vi "bats.parser.generated.vi"(9 "time":u64, 10 "data.stream":T1={"data"=[0, 0, 0, 0, 0, 0, 0, 0], "data valid"=FALSE, "byte enables"=[FALSE, FALSE, FALSE, FALSE, FALSE, FALSE, FALSE, FALSE], "eof.good"=FALSE, "eof.bad"=FALSE, "recv.time"=0}, 11 "reset":bool) -> (2 "Ready.for.Udp.Input":bool)   [LabVIEW 2020]
doc: "REFERENCE COPY of bats.parser.vi, built 2026-10-14 from its AIXML export. The two FPGA FIFO Write nodes (handshake interface), which AIXML cannot carry, are replaced by calls to FIFO.WRITE.vi with the FIFO's configuration wired as constants: FIFO Name and Data Type, Element through To Variant. Everything else is the exported diagram; typedefs come back as bare clusters (rebind if this is ever used for real). To put the real FIFO nodes back: replace each FIFO.WRITE.vi call with the FPGA FIFO Method Node (Write) for the named FIFO, wire Element and Input Valid, read Ready for Input, delete the constants and To Variant."
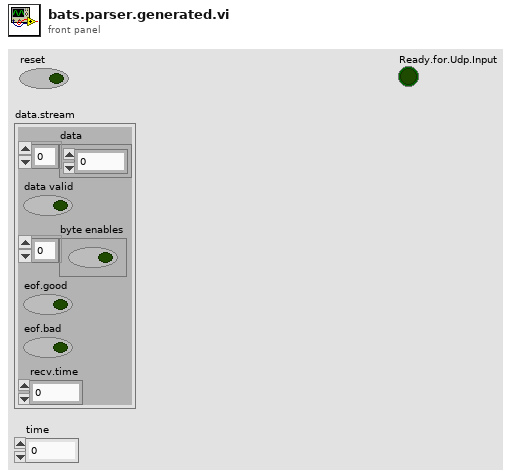
[diagram p1: front panel]
types:
  T1 = cluster{"data":u8[], "data valid":bool, "byte enables":bool[], "eof.good":bool, "eof.bad":bool, "recv.time":u64}
  T2 = cluster{"reset":bool, "data.stream":cluster{"data":u8[], "data valid":bool, "byte enables":bool[], "eof.good":bool, "eof.bad":bool, "recv.time":u64}}
  T3 = enum16{"Reset", "Noop", "Read.Sequenced.Unit.Header", "Read.Msg"}
  T4 = cluster{"BATS.Parser.States":enum16{"Reset", "Noop", "Read.Sequenced.Unit.Header", "Read.Msg"}, "Saved.BATS.Parser.State":enum16{"Reset", "Noop", "Read.Sequenced.Unit.Header", "Read.Msg"}, "Hdr Length (U16)":u16, "MessageLength (U8)":u8, "MessageType (U8)":u8, "Time (U32)":u32, "Total Counter (U16)":u16, "Message Counter (U8)":u8, "i":u16, "Number.of.Tickers":u16, "n":u16, "msg.counter":u8, "msg.length":u8, "buffer.start":u8, "buffer.length":u8, "buffer":u64[], "Next.Seq.No":u32, "debug":cluster{"write":bool, "data":u64[]}}
  T5 = enum8{"Time", "AddOrder", "OrderExecuted", "OrderExecutedAtPrice", "ReduceSize", "ModifyOrder", "DeleteOrder", "Get.Everything", "Get.All.Orders", "Get.Top", "Trade", "Unsupported"}
  T6 = cluster{"type":enum8{"Time", "AddOrder", "OrderExecuted", "OrderExecutedAtPrice", "ReduceSize", "ModifyOrder", "DeleteOrder", "Get.Everything", "Get.All.Orders", "Get.Top", "Trade", "Unsupported"}, "side":u8, "orderId ":u64, "quantity":u32, "symbol":u64, "price":u64, "executed.qty":u32, "canceled.qty":u32, "remaining.qty":u32, "seconds":u64, "nanoseconds":u64, "Add":bool, "Edit":bool, "Remove":bool, "seq no":u32, "recv.time":u64, "parse.time":u64}
  T7 = typedef "fpganow.common.fpga.lvlib/orderbook.command.ctl" = cluster{"type":T8, "side":u8, "orderId ":u64, "quantity":u32, "symbol":u64, "price":u64, "executed.qty":u32, "canceled.qty":u32, "remaining.qty":u32, "seconds":u64, "nanoseconds":u64, "Add":bool, "Edit":bool, "Remove":bool, "seq no":u32, "recv.time":u64, "parse.time":u64}
  T8 = typedef "fpganow.common.fpga.lvlib/orderbook.command.type.ctl" = enum8{"Time", "AddOrder", "OrderExecuted", "OrderExecutedAtPrice", "ReduceSize", "ModifyOrder", "DeleteOrder", "Get.Everything", "Get.All.Orders", "Get.Top", "Trade", "Unsupported"}
  T9 = cluster{"type":enum8{"Time", "AddOrder", "OrderExecuted", "OrderExecutedAtPrice", "ReduceSize", "ModifyOrder", "DeleteOrder", "Get.Everything", "Get.All.Orders", "Get.Top"}, "side":u8, "orderId ":u64, "quantity":u32, "symbol":u64, "price":u64, "executed.qty":u32, "canceled.qty":u32, "remaining.qty":u32, "seconds":u64, "nanoseconds":u64, "Add":bool, "Edit":bool, "Remove":bool, "seq no":u32, "recv.time":u64, "parse.time":u64}
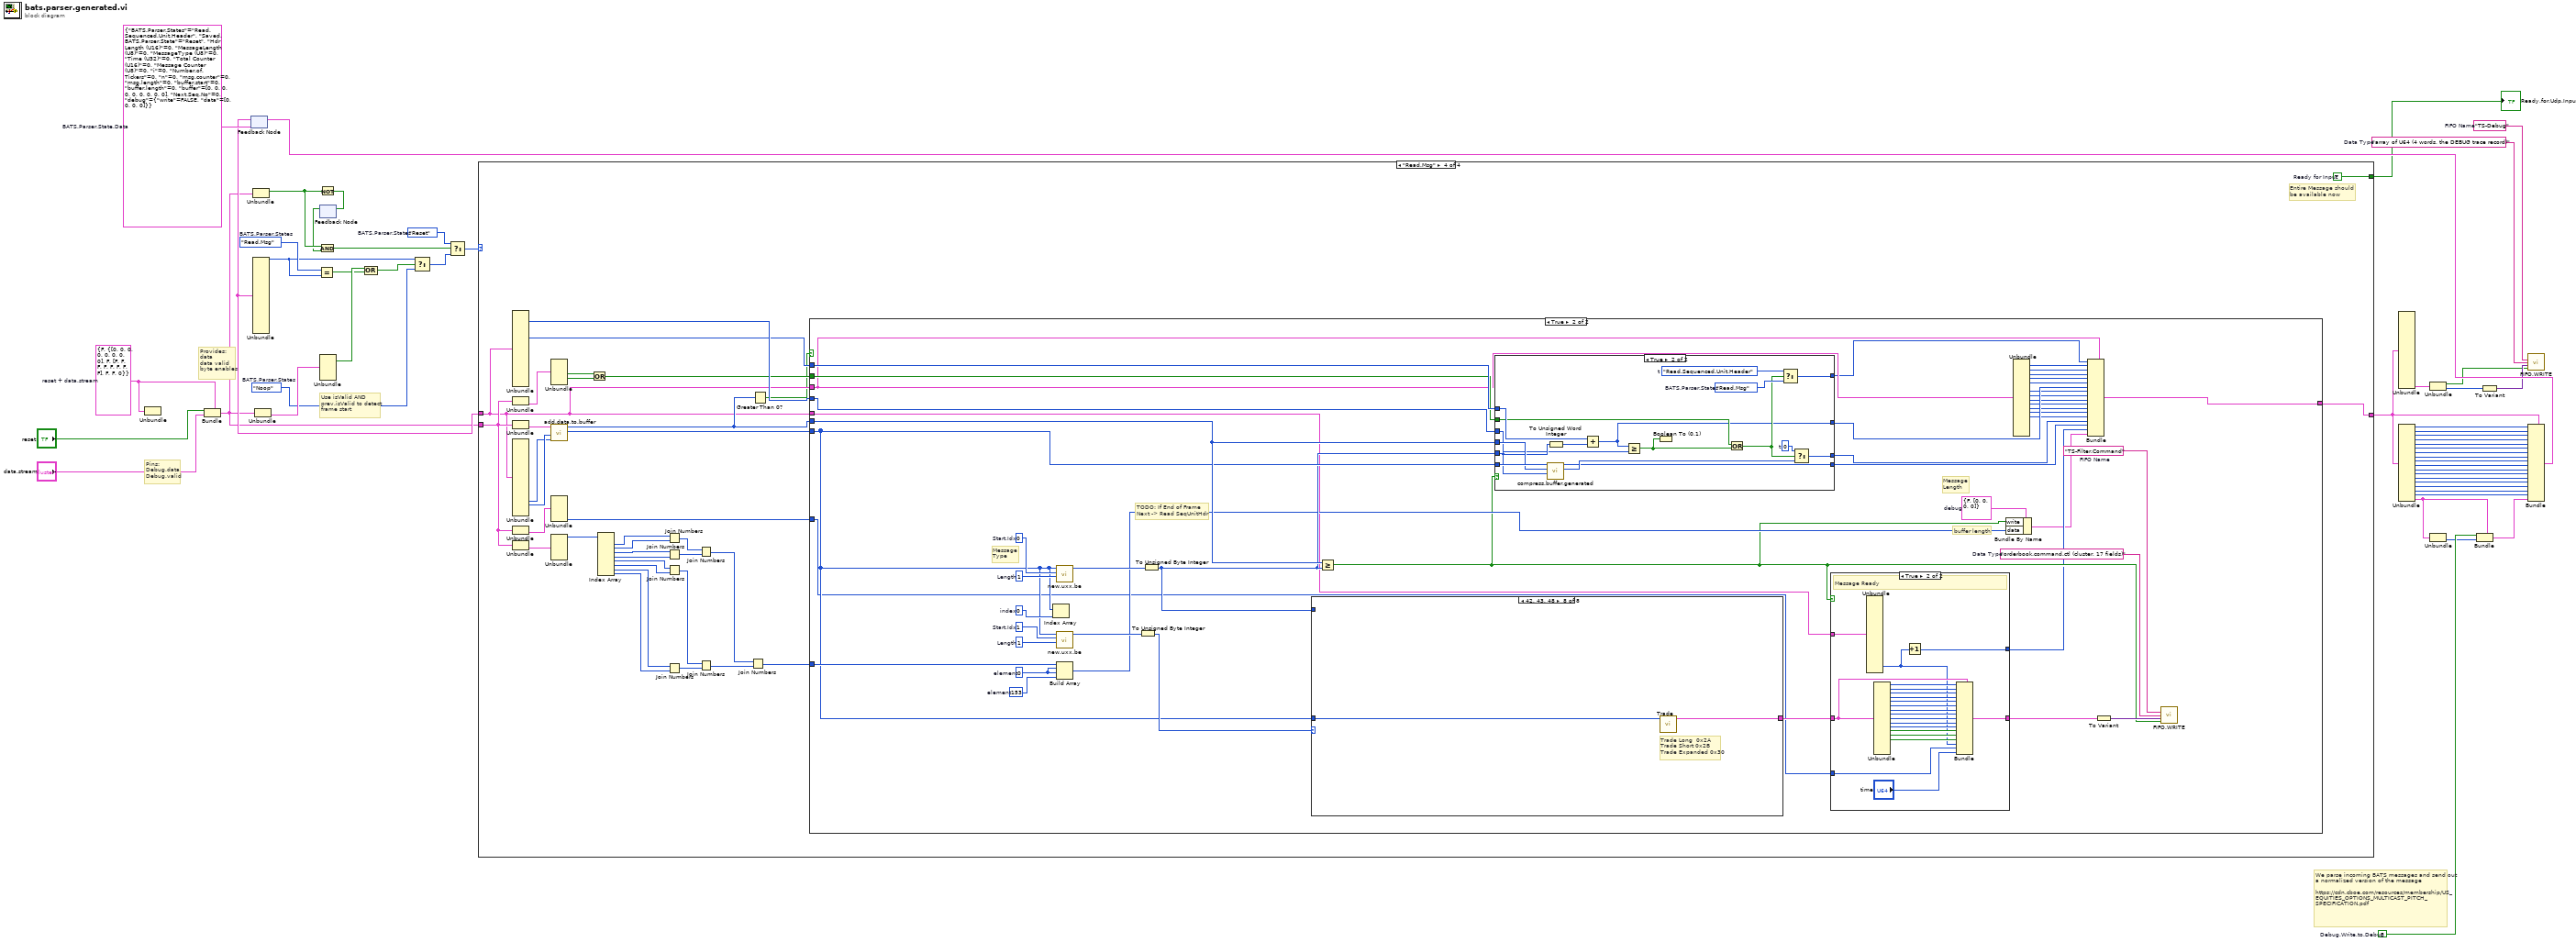
[diagram p0: block diagram]
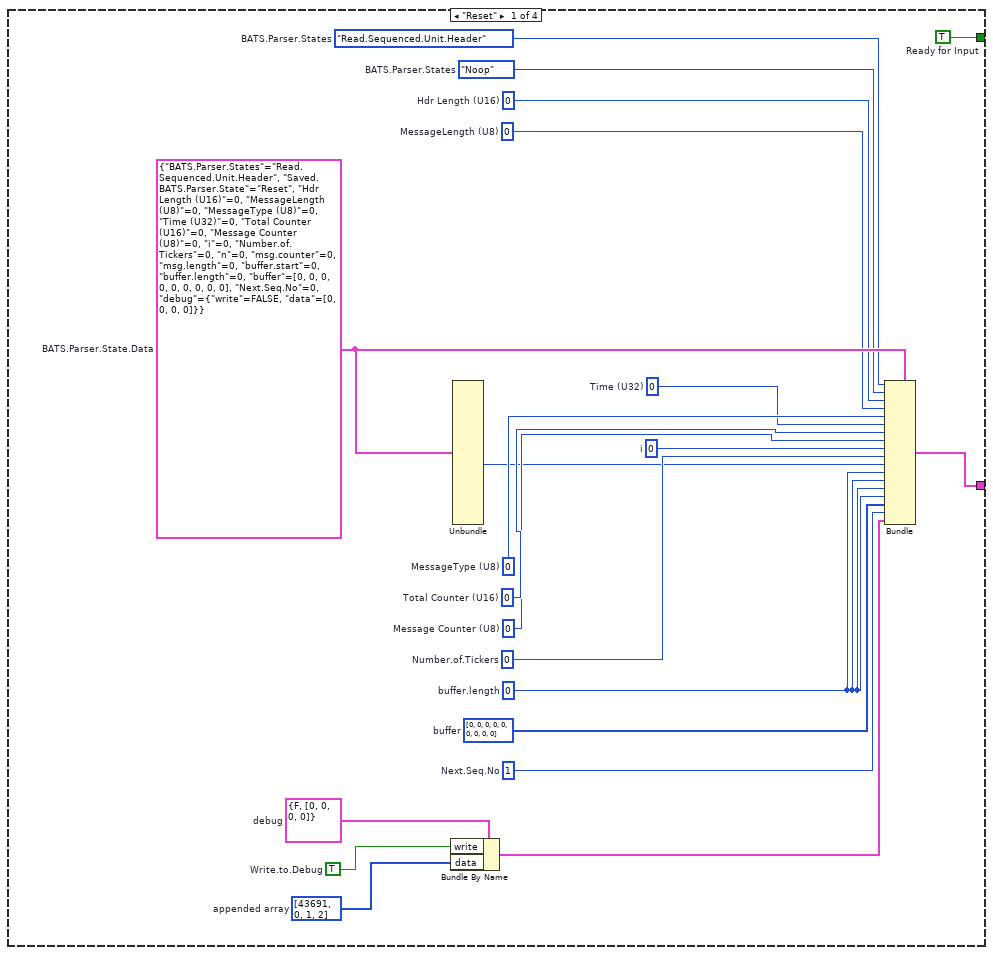
[diagram p2: hidden frame]
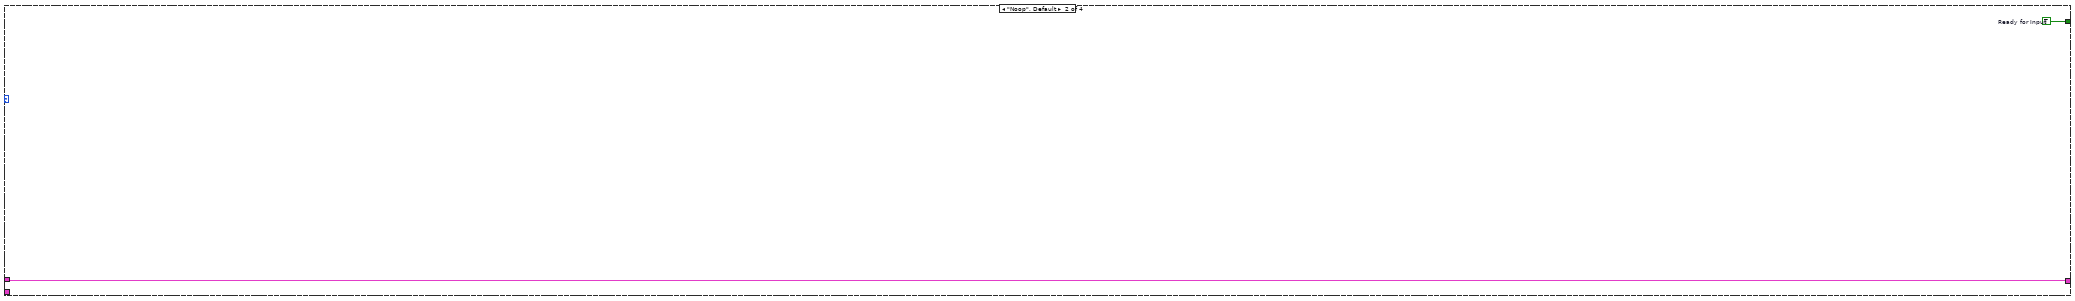
[diagram p3: hidden frame]
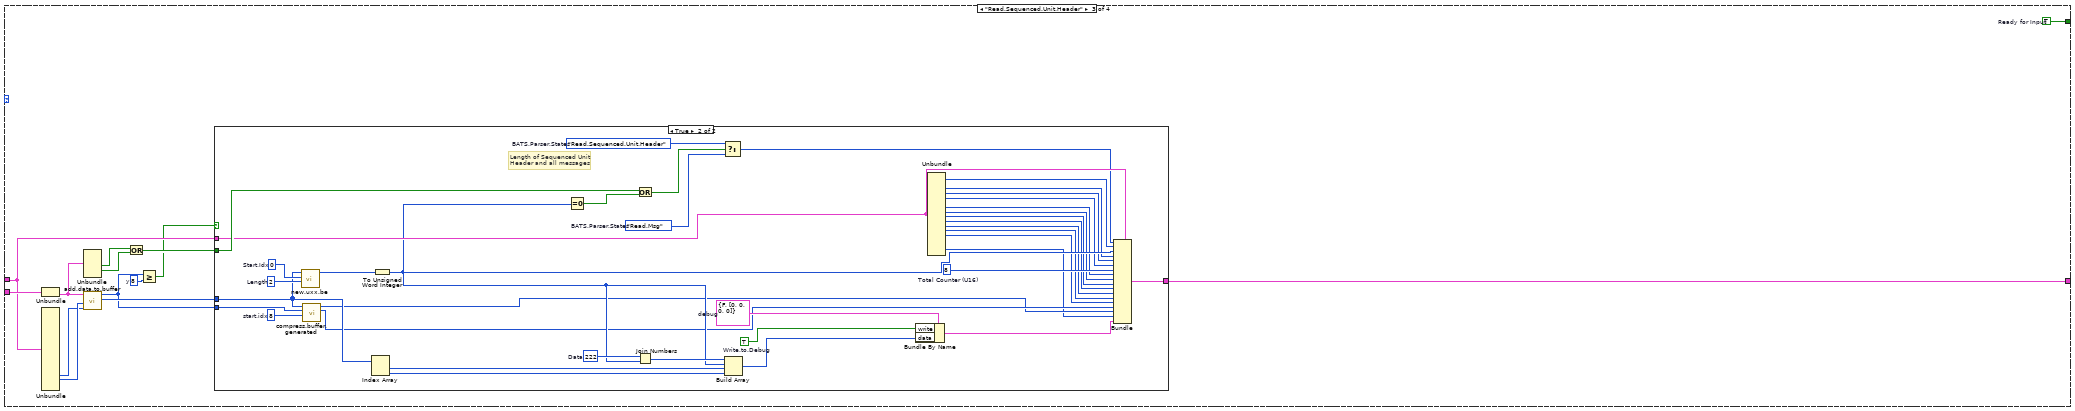
[diagram p4: hidden frame]
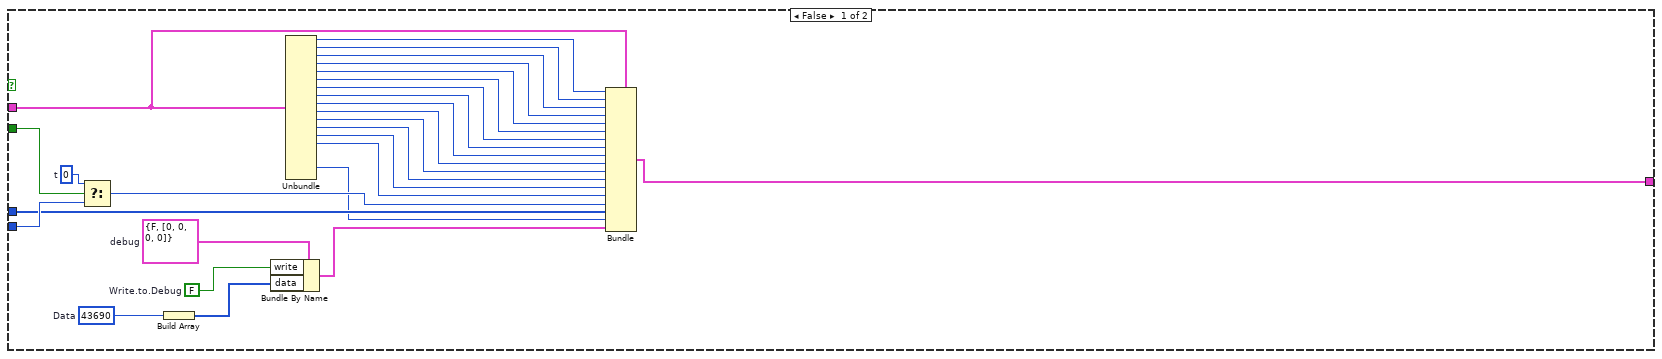
[diagram p5: hidden frame]
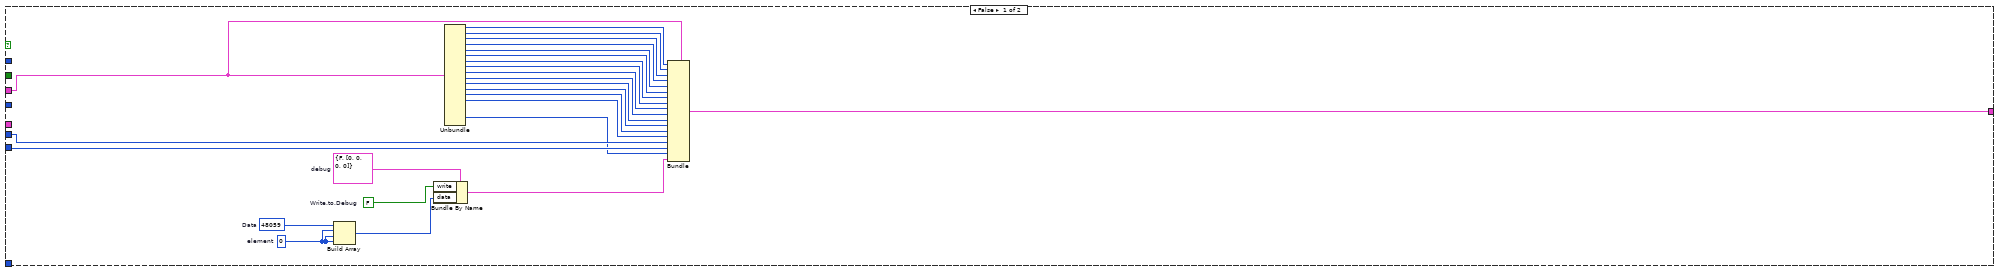
[diagram p6: hidden frame]
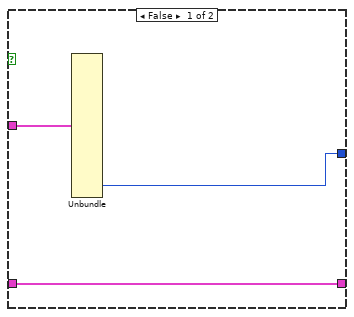
[diagram p7: hidden frame]
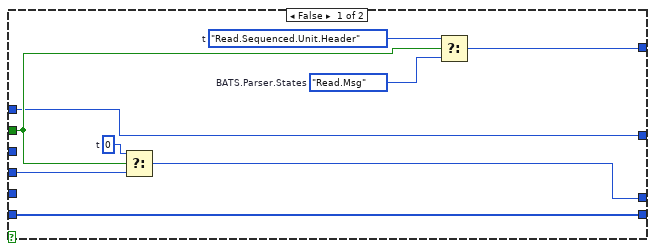
[diagram p8: hidden frame]
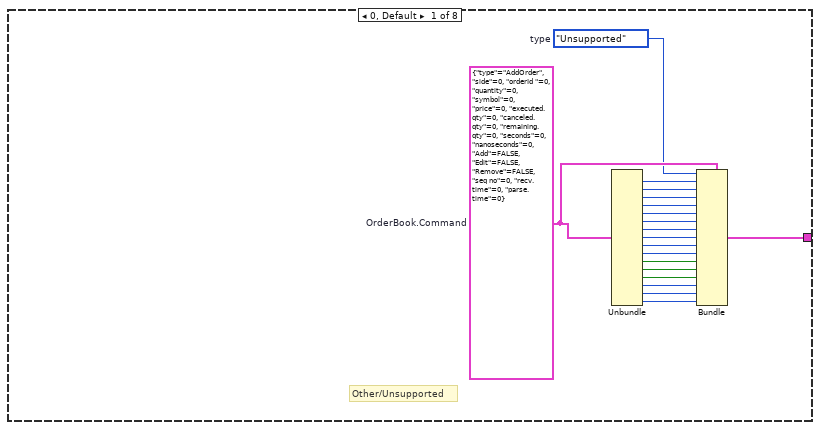
[diagram p9: hidden frame]
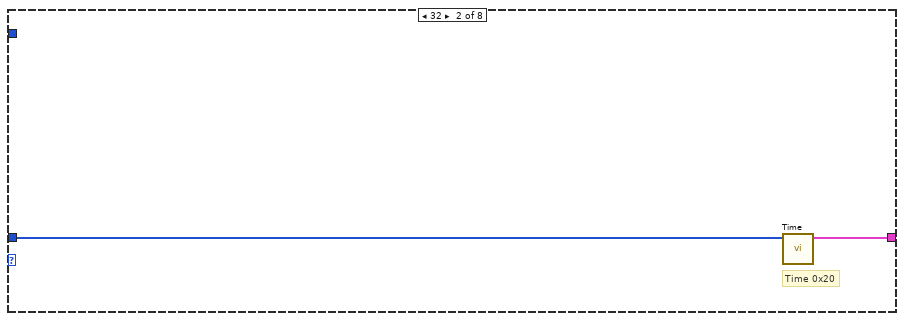
[diagram p10: hidden frame]
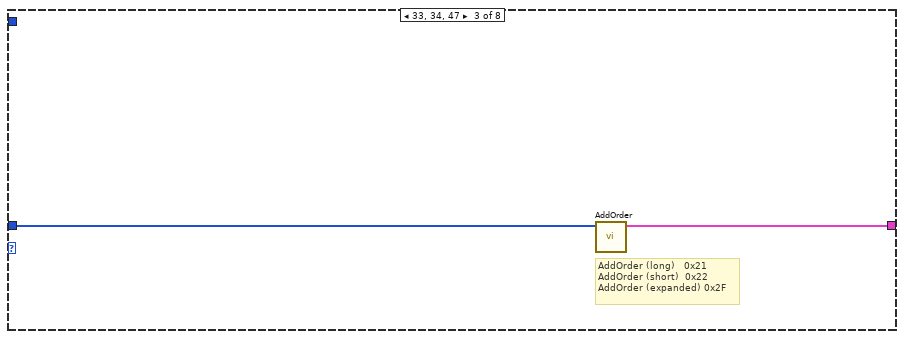
[diagram p11: hidden frame]
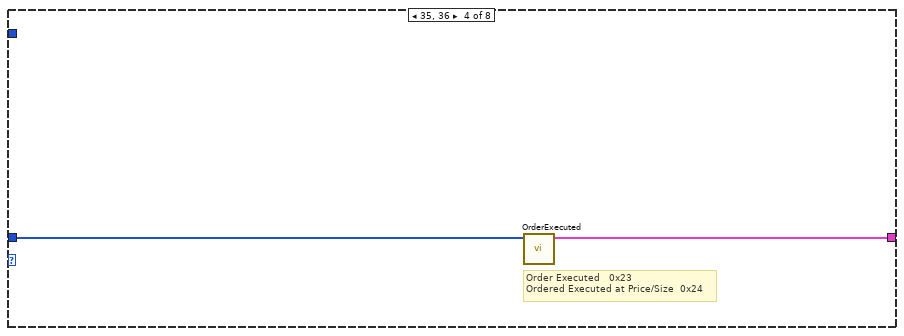
[diagram p12: hidden frame]
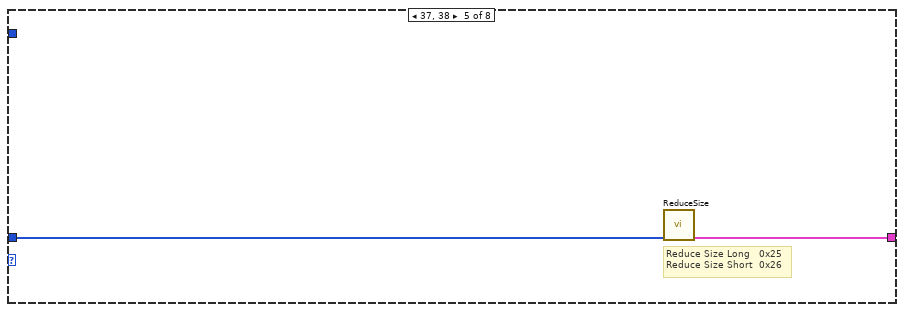
[diagram p13: hidden frame]
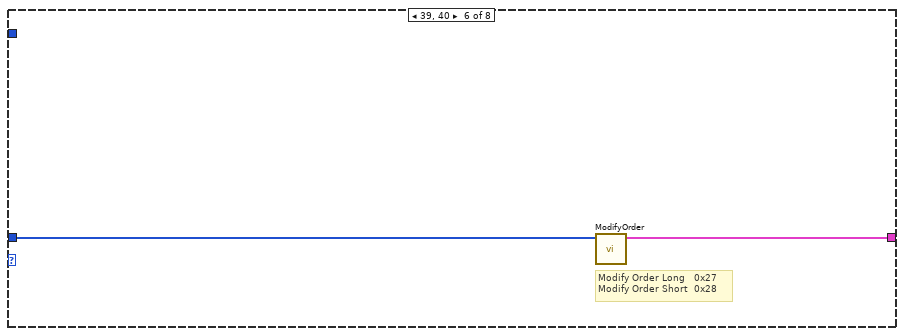
[diagram p14: hidden frame]
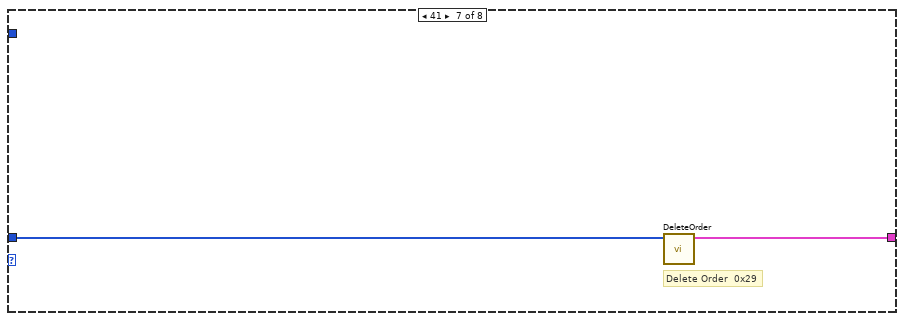
[diagram p15: hidden frame]
diagram:
  w4 = "array of U64 (4 words, the DEBUG trace record)"  # Data Type
  w5 = "TS-Debug"  # FIFO Name
  w49 = T2 {"reset"=FALSE, "data.stream"={"data"=[0, 0, 0, 0, 0, 0, 0, 0], "data valid"=FALSE, "byte enables"=[FALSE, FALSE, FALSE, FALSE, FALSE, FALSE, FALSE, FALSE], "eof.good"=FALSE, "eof.bad"=FALSE, "recv.time"=0}}  # reset + data.stream
  w29 = FALSE  # Debug.Write.to.Debug
  w45 = T3."Read.Msg"  # BATS.Parser.States
  w36 = T3."Reset"  # BATS.Parser.States
  w37 = T3."Noop"  # BATS.Parser.States
  w50 = T4 {"BATS.Parser.States"=enum."Read.Sequenced.Unit.Header", "Saved.BATS.Parser.State"=enum."Reset", "Hdr Length (U16)"=0, "MessageLength (U8)"=0, "MessageType (U8)"=0, "Time (U32)"=0, "Total Counter (U16)"=0, "Message Counter (U8)"=0, "i"=0, "Number.of.Tickers"=0, "n"=0, "msg.counter"=0, "msg.length"=0, "buffer.start"=0, "buffer.length"=0, "buffer"=[0, 0, 0, 0, 0, 0, 0, 0, 0], "Next.Seq.No"=0, "debug"={"write"=FALSE, "data"=[0, 0, 0, 0]}}  # BATS.Parser.State.Data
  # "We parse incoming BATS messages and send out\na normalized version of the message\n\nhttps://cdn.cboe.com/resources/membership/US_EQUITIES_OPTIONS_MULTICAST_PITCH_SPECIFICATION.pdf"
  # "Pins:\nDebug.data\nDebug.valid"
  # "Provides:\ndata\ndata valid\nbyte enables"
  # "Use isValid AND\nprev.isValid to detect\nframe start"
  n1 = Unbundle(w49) -> ()  [unwired: 2 out]
  n2 = Bundle(cluster=w49, "reset"="reset", "data.stream"="data.stream") -> (w32:T2)
  n3 = feedback #1(w50) -> (w33:T4)
  n4 = Unbundle(w32) -> ("reset"=w43:bool)  [unwired: 1 out]
  n5 = Unbundle(w33) -> ("BATS.Parser.States"=w39:T3)  [unwired: 17 out]
  n6 = Unbundle(w32) -> ("data.stream"=w46:T1)  [unwired: 1 out]
  n7 = Equal?(x=w45, y=w39) -> (x = y?=w40:bool)
  n8 = Not(x=w43) -> (.not. x?=w44:bool)
  n9 = feedback-in #2(w44) -> ()
  n10 = feedback #2() -> (w42:bool)  [unwired: 1 in]
  n11 = And(x=w43, y=w42) -> (x .and. y?=w35:bool)
  n12 = Unbundle(w46) -> ("data valid"=w41:bool)  [unwired: 5 out]
  n13 = Compound Arithmetic op=OR(w41, w40) -> (w38:bool)
  n14 = Select(t=w39, s=w38, f=w37) -> (s? t:f=w34:T3)
  n15 = Select(t=w36, s=w35, f=w34) -> (s? t:f=w31:T3)
  n16 = case shown="\"Read.Msg\"" w31 {
    tunnel: w33 -> [_ w73 w78 w159]
    tunnel: w32 -> [_ _ w87 w185]
    tunnel: [w52 w73 w75 w154] -> w8
    tunnel: [w51 w72 w74 w153] -> w1
    frame "Reset" {
      w70 = u64[] [43691, 0, 1, 2]  # appended array
      w69 = cluster{"write":bool, "data":u64[]} {"write"=FALSE, "data"=[0, 0, 0, 0]}  # debug
      w54 = u32 1  # Next.Seq.No
      w51 = TRUE  # Ready for Input
      w67 = T3."Read.Sequenced.Unit.Header"  # BATS.Parser.States
      w71 = TRUE  # Write.to.Debug
      w56 = u8 0  # buffer.length
      w55 = u64[] [0, 0, 0, 0, 0, 0, 0, 0, 0]  # buffer
      w58 = u16 0  # Number.of.Tickers
      w59 = u16 0  # i
      w60 = u8 0  # Message Counter (U8)
      w61 = u16 0  # Total Counter (U16)
      w62 = u32 0  # Time (U32)
      w63 = u8 0  # MessageType (U8)
      w64 = u8 0  # MessageLength (U8)
      w65 = u16 0  # Hdr Length (U16)
      w66 = T3."Noop"  # BATS.Parser.States
      w68 = T4 {"BATS.Parser.States"=enum."Read.Sequenced.Unit.Header", "Saved.BATS.Parser.State"=enum."Reset", "Hdr Length (U16)"=0, "MessageLength (U8)"=0, "MessageType (U8)"=0, "Time (U32)"=0, "Total Counter (U16)"=0, "Message Counter (U8)"=0, "i"=0, "Number.of.Tickers"=0, "n"=0, "msg.counter"=0, "msg.length"=0, "buffer.start"=0, "buffer.length"=0, "buffer"=[0, 0, 0, 0, 0, 0, 0, 0, 0], "Next.Seq.No"=0, "debug"={"write"=FALSE, "data"=[0, 0, 0, 0]}}  # BATS.Parser.State.Data
      n17 = Bundle By Name(cluster=w69, "write"=w71, "data"=w70) -> (w53:cluster{"write":bool, "data":u64[]})
      n18 = Unbundle(w68) -> ("n"=w57:u16)  [unwired: 17 out]
      n19 = Bundle(cluster=w68, "BATS.Parser.States"=w67, "Saved.BATS.Parser.State"=w66, "Hdr Length (U16)"=w65, "MessageLength (U8)"=w64, "MessageType (U8)"=w63, "Time (U32)"=w62, "Total Counter (U16)"=w61, "Message Counter (U8)"=w60, "i"=w59, "Number.of.Tickers"=w58, "n"=w57, "msg.counter"=w56, "msg.length"=w56, "buffer.start"=w56, "buffer.length"=w56, "buffer"=w55, "Next.Seq.No"=w54, "debug"=w53) -> (w52:T4)
    }
    frame "Noop", Default {
      w72 = TRUE  # Ready for Input
    }
    frame "Read.Sequenced.Unit.Header" {
      w74 = TRUE  # Ready for Input
      w83 = u8 8  # y
      n20 = Unbundle(w87) -> ("data.stream"=w84:T1)  [unwired: 1 out]
      n21 = Unbundle(w78) -> ("buffer.length"=w85:u8, "buffer"=w86:u64[])  [unwired: 16 out]
      n22 = Unbundle(w84) -> ("eof.good"=w82:bool, "eof.bad"=w81:bool)  [unwired: 4 out]
      n23 = call "add.data.to.buffer.vi"("buffer.length"=w85, "buffer"=w86, "data.stream"=w84) -> ("buffer.out"=w80:u64[], "buffer.length.out"=w79:u8)  [unwired: 7 in]
      n24 = Or(x=w82, y=w81) -> (x .or. y?=w77:bool)
      n25 = Greater Or Equal?(x=w79, y=w83) -> (x >= y?=w76:bool)
      n26 = case shown="True" w76 {
        tunnel: w80 -> [w91 w150]
        tunnel: w79 -> [w111 w149]
        tunnel: w78 -> [w107 w134]
        tunnel: w77 -> [w112 w142]
        tunnel: [w88 w115] -> w75
        frame False {
          w113 = u8 0  # t
          w108 = cluster{"write":bool, "data":u64[]} {"write"=FALSE, "data"=[0, 0, 0, 0]}  # debug
          w114 = u64 43690  # Data
          w110 = FALSE  # Write.to.Debug
          n27 = Select(t=w113, s=w112, f=w111) -> (s? t:f=w92:u8)
          n28 = Build Array(w114) -> (w109:u64[])
          n29 = Bundle By Name(cluster=w108, "write"=w110, "data"=w109) -> (w89:cluster{"write":bool, "data":u64[]})
          n30 = Unbundle(w107) -> ("BATS.Parser.States"=w106:T3, "Saved.BATS.Parser.State"=w105:T3, "Hdr Length (U16)"=w104:u16, "MessageLength (U8)"=w103:u8, "MessageType (U8)"=w102:u8, "Time (U32)"=w101:u32, "Total Counter (U16)"=w100:u16, "Message Counter (U8)"=w99:u8, "i"=w98:u16, "Number.of.Tickers"=w97:u16, "n"=w96:u16, "msg.counter"=w95:u8, "msg.length"=w94:u8, "buffer.start"=w93:u8, "Next.Seq.No"=w90:u32)  [unwired: 3 out]
          n31 = Bundle(cluster=w107, "BATS.Parser.States"=w106, "Saved.BATS.Parser.State"=w105, "Hdr Length (U16)"=w104, "MessageLength (U8)"=w103, "MessageType (U8)"=w102, "Time (U32)"=w101, "Total Counter (U16)"=w100, "Message Counter (U8)"=w99, "i"=w98, "Number.of.Tickers"=w97, "n"=w96, "msg.counter"=w95, "msg.length"=w94, "buffer.start"=w93, "buffer.length"=w92, "buffer"=w91, "Next.Seq.No"=w90, "debug"=w89) -> (w88:T4)
        }
        frame True {
          w135 = T3."Read.Msg"  # BATS.Parser.States
          w138 = cluster{"write":bool, "data":u64[]} {"write"=FALSE, "data"=[0, 0, 0, 0]}  # debug
          w146 = u32 222  # Data
          w127 = u16 8  # Total Counter (U16)
          w140 = TRUE  # Write.to.Debug
          w148 = u8 8  # start.idx
          w151 = u8 2  # Length
          w152 = u8 0  # Start.Idx
          w137 = T3."Read.Sequenced.Unit.Header"  # BATS.Parser.States
          # "Length of Sequenced Unit\nHeader and all messages"
          n32 = call "new.uxx.be.vi"("buffer (U64)"=w150, "Start.Idx"=w152, "Length"=w151) -> ("Out.Value U64"=w147:u64)  [unwired: 7 in]
          n33 = call "compress.buffer.generated.vi"("start.idx"=w148, "buffer.length"=w149, "buffer"=w150) -> ("buffer.length.out"=w119:u8, "buffer.out"=w118:u64[])  [unwired: 7 in]
          n34 = Index Array(array=w150) -> (element #1=w144:u64, element #2=w143:u64)  [unwired: 2 in]
          n35 = To Unsigned Word Integer(number=w147) -> (unsigned 16bit integer=w131:u16)
          n36 = Equal To 0?(x=w131) -> (x = 0?=w141:bool)
          n37 = Or(x=w142, y=w141) -> (x .or. y?=w136:bool)
          n38 = Join Numbers(hi=w146, lo=w131) -> ((hi.lo)=w145:u64)
          n39 = Select(t=w137, s=w136, f=w135) -> (s? t:f=w133:T3)
          n40 = Build Array(w145, w131, w144, w143) -> (w139:u64[])
          n41 = Bundle By Name(cluster=w138, "write"=w140, "data"=w139) -> (w116:cluster{"write":bool, "data":u64[]})
          n42 = Unbundle(w134) -> ("Saved.BATS.Parser.State"=w132:T3, "MessageLength (U8)"=w130:u8, "MessageType (U8)"=w129:u8, "Time (U32)"=w128:u32, "Message Counter (U8)"=w126:u8, "i"=w125:u16, "Number.of.Tickers"=w124:u16, "n"=w123:u16, "msg.counter"=w122:u8, "msg.length"=w121:u8, "buffer.start"=w120:u8, "Next.Seq.No"=w117:u32)  [unwired: 6 out]
          n43 = Bundle(cluster=w134, "BATS.Parser.States"=w133, "Saved.BATS.Parser.State"=w132, "Hdr Length (U16)"=w131, "MessageLength (U8)"=w130, "MessageType (U8)"=w129, "Time (U32)"=w128, "Total Counter (U16)"=w127, "Message Counter (U8)"=w126, "i"=w125, "Number.of.Tickers"=w124, "n"=w123, "msg.counter"=w122, "msg.length"=w121, "buffer.start"=w120, "buffer.length"=w119, "buffer"=w118, "Next.Seq.No"=w117, "debug"=w116) -> (w115:T4)
        }
      }
    }
    frame "Read.Msg" {
      w153 = TRUE  # Ready for Input
      # "Entire Message should \nbe available now"
      n44 = Unbundle(w159) -> ("Hdr Length (U16)"=w161:u16, "Total Counter (U16)"=w160:u16)  [unwired: 16 out]
      n45 = Unbundle(w185) -> ("data.stream"=w184:T1)  [unwired: 1 out]
      n46 = Unbundle(w185) -> ("data.stream"=w182:T1)  [unwired: 1 out]
      n47 = Unbundle(w159) -> ("buffer.length"=w180:u8, "buffer"=w181:u64[])  [unwired: 16 out]
      n48 = Unbundle(w185) -> ("data.stream"=w186:T1)  [unwired: 1 out]
      n49 = Unbundle(w185) -> ("data.stream"=w187:T1)  [unwired: 1 out]
      n50 = Unbundle(w184) -> ("eof.good"=w179:bool, "eof.bad"=w178:bool)  [unwired: 4 out]
      n51 = call "add.data.to.buffer.vi"("buffer.length"=w180, "buffer"=w181, "data.stream"=w182) -> ("buffer.out"=w163:u64[], "buffer.length.out"=w162:u8)  [unwired: 7 in]
      n52 = Unbundle(w186) -> ("recv.time"=w157:u64)  [unwired: 5 out]
      n53 = Unbundle(w187) -> ("data"=w183:u8[])  [unwired: 5 out]
      n54 = Or(x=w179, y=w178) -> (x .or. y?=w156:bool)
      n55 = Index Array(array=w183) -> (element #1=w177:u8, element #2=w176:u8, element #3=w175:u8, element #4=w174:u8, element #5=w173:u8, element #6=w172:u8, element #7=w171:u8, element #8=w170:u8)  [unwired: 8 in]
      n56 = Join Numbers(hi=w177, lo=w176) -> ((hi.lo)=w169:u16)
      n57 = Join Numbers(hi=w175, lo=w174) -> ((hi.lo)=w168:u16)
      n58 = Join Numbers(hi=w173, lo=w172) -> ((hi.lo)=w167:u16)
      n59 = Join Numbers(hi=w171, lo=w170) -> ((hi.lo)=w166:u16)
      n60 = Join Numbers(hi=w169, lo=w168) -> ((hi.lo)=w165:u32)
      n61 = Join Numbers(hi=w167, lo=w166) -> ((hi.lo)=w164:u32)
      n62 = Join Numbers(hi=w165, lo=w164) -> ((hi.lo)=w158:u64)
      n63 = Greater Than 0?(x=w162) -> (x > 0?=w155:bool)
      n64 = case shown="True" w155 {
        tunnel: w163 -> [w191 w247]
        tunnel: w162 -> [w192 w248]
        tunnel: w159 -> [w207 w232]
        tunnel: w161 -> [_ w245]
        tunnel: w160 -> [_ w244]
        tunnel: w159 -> [_ w239]
        tunnel: w158 -> [_ w254]
        tunnel: w157 -> [_ w238]
        tunnel: w156 -> [_ w243]
        tunnel: [w188 w213] -> w154
        frame False {
          w211 = u64 0  # element
          w208 = cluster{"write":bool, "data":u64[]} {"write"=FALSE, "data"=[0, 0, 0, 0]}  # debug
          w212 = u64 48059  # Data
          w210 = FALSE  # Write.to.Debug
          n65 = Build Array(w212, w211, w211, w211) -> (w209:u64[])
          n66 = Bundle By Name(cluster=w208, "write"=w210, "data"=w209) -> (w189:cluster{"write":bool, "data":u64[]})
          n67 = Unbundle(w207) -> ("BATS.Parser.States"=w206:T3, "Saved.BATS.Parser.State"=w205:T3, "Hdr Length (U16)"=w204:u16, "MessageLength (U8)"=w203:u8, "MessageType (U8)"=w202:u8, "Time (U32)"=w201:u32, "Total Counter (U16)"=w200:u16, "Message Counter (U8)"=w199:u8, "i"=w198:u16, "Number.of.Tickers"=w197:u16, "n"=w196:u16, "msg.counter"=w195:u8, "msg.length"=w194:u8, "buffer.start"=w193:u8, "Next.Seq.No"=w190:u32)  [unwired: 3 out]
          n68 = Bundle(cluster=w207, "BATS.Parser.States"=w206, "Saved.BATS.Parser.State"=w205, "Hdr Length (U16)"=w204, "MessageLength (U8)"=w203, "MessageType (U8)"=w202, "Time (U32)"=w201, "Total Counter (U16)"=w200, "Message Counter (U8)"=w199, "i"=w198, "Number.of.Tickers"=w197, "n"=w196, "msg.counter"=w195, "msg.length"=w194, "buffer.start"=w193, "buffer.length"=w192, "buffer"=w191, "Next.Seq.No"=w190, "debug"=w189) -> (w188:T4)
        }
        frame True {
          w235 = "orderbook.command.ctl (cluster, 17 fields)"  # Data Type
          w236 = "TS-Filter.Command"  # FIFO Name
          w253 = u64 0  # element
          w252 = u64 153  # element
          w241 = cluster{"write":bool, "data":u64[]} {"write"=FALSE, "data"=[0, 0, 0, 0]}  # debug
          w255 = 0  # index
          w256 = u8 1  # Length
          w257 = u8 1  # Start.Idx
          w258 = u8 1  # Length
          w259 = u8 0  # Start.Idx
          # "Message\nLength"
          # "Message\nType"
          # "buffer length"
          # "TODO: If End of Frame\nNext -> Read SeqUnitHdr"
          n69 = Index Array(array=w247, index=w255) -> ()  [unwired: 1 out]
          n70 = call "new.uxx.be.vi"("buffer (U64)"=w247, "Start.Idx"=w259, "Length"=w258) -> ("Out.Value U64"=w251:u64)  [unwired: 7 in]
          n71 = call "new.uxx.be.vi"("buffer (U64)"=w247, "Start.Idx"=w257, "Length"=w256) -> ("Out.Value U64"=w250:u64)  [unwired: 7 in]
          n72 = Build Array(w254, w253, w253, w252) -> (w242:u64[])
          n73 = To Unsigned Byte Integer(number=w250) -> (unsigned 8bit integer=w249:u8)
          n74 = To Unsigned Byte Integer(number=w251) -> (unsigned 8bit integer=w246:u8)
          n75 = case shown="42, 43, 48" w249 {
            tunnel: w247 -> [_ w330 w332 w334 w336 w338 w340 w342]
            tunnel: w246 -> [_ _ _ _ _ _ _ _]
            tunnel: [w310 w329 w331 w333 w335 w337 w339 w341] -> w240
            frame 0, Default {
              w327 = T5."Unsupported"  # type
              w328 = T6 {"type"=enum."AddOrder", "side"=0, "orderId "=0, "quantity"=0, "symbol"=0, "price"=0, "executed.qty"=0, "canceled.qty"=0, "remaining.qty"=0, "seconds"=0, "nanoseconds"=0, "Add"=FALSE, "Edit"=FALSE, "Remove"=FALSE, "seq no"=0, "recv.time"=0, "parse.time"=0}  # OrderBook.Command
              # "Other/Unsupported"
              n76 = Unbundle(w328) -> ("side"=w326:u8, "orderId"=w325:u64, "quantity"=w324:u32, "symbol"=w323:u64, "price"=w322:u64, "executed.qty"=w321:u32, "canceled.qty"=w320:u32, "remaining.qty"=w319:u32, "seconds"=w318:u64, "nanoseconds"=w317:u64, "Add"=w316:bool, "Edit"=w315:bool, "Remove"=w314:bool, "seq no"=w313:u32, "recv.time"=w312:u64, "parse.time"=w311:u64)  [unwired: 1 out]
              n77 = Bundle(cluster=w328, "type"=w327, "side"=w326, "orderId"=w325, "quantity"=w324, "symbol"=w323, "price"=w322, "executed.qty"=w321, "canceled.qty"=w320, "remaining.qty"=w319, "seconds"=w318, "nanoseconds"=w317, "Add"=w316, "Edit"=w315, "Remove"=w314, "seq no"=w313, "recv.time"=w312, "parse.time"=w311) -> (w310:T6)
            }
            frame 32 {
              # "Time 0x20"
              n78 = call "Time.vi"("buffer.in"=w330) -> ("OrderBook.Command"=w329:T7)  [unwired: 10 in]
            }
            frame 33, 34, 47 {
              # "AddOrder (long)   0x21\nAddOrder (short)  0x22\nAddOrder (expanded) 0x2F"
              n79 = call "AddOrder.vi"("buffer.in"=w332) -> ("OrderBook.Command"=w331:T7)  [unwired: 10 in]
            }
            frame 35, 36 {
              # "Order Executed   0x23\nOrdered Executed at Price/Size  0x24"
              n80 = call "OrderExecuted.vi"("buffer.in"=w334) -> ("OrderBook.Command"=w333:T7)  [unwired: 10 in]
            }
            frame 37, 38 {
              # "Reduce Size Long   0x25\nReduce Size Short  0x26"
              n81 = call "ReduceSize.vi"("buffer.in"=w336) -> ("orderbook.command"=w335:T7)  [unwired: 14 in]
            }
            frame 39, 40 {
              # "Modify Order Long   0x27\nModify Order Short  0x28"
              n82 = call "ModifyOrder.vi"("buffer.in"=w338) -> ("OrderBook.Command"=w337:T9)  [unwired: 10 in]
            }
            frame 41 {
              # "Delete Order  0x29"
              n83 = call "DeleteOrder.vi"("buffer.in"=w340) -> ("OrderBook.Command"=w339:T9)  [unwired: 10 in]
            }
            frame 42, 43, 48 {
              # "Trade Long  0x2A\nTrade Short 0x2B\nTrade Expanded 0x30"
              n84 = call "Trade.vi"("buffer.in"=w342) -> ("OrderBook.Command"=w341:T6)  [unwired: 10 in]
            }
          }
          n85 = Greater Or Equal?(x=w248, y=w246) -> (x >= y?=w233:bool)
          n86 = case shown="True" w233 {
            tunnel: w248 -> [w288 w308]
            tunnel: w247 -> [w286 w309]
            tunnel: w246 -> [_ w307]
            tunnel: w245 -> [_ w304]
            tunnel: w244 -> [w284 w306]
            tunnel: w243 -> [w289 w303]
            tunnel: [w287 w296] -> w217
            tunnel: [w286 w295] -> w216
            tunnel: [w285 w294] -> w231
            tunnel: [w284 w293] -> w225
            frame False {
              w290 = u8 0  # t
              w292 = T3."Read.Sequenced.Unit.Header"  # t
              w291 = T3."Read.Msg"  # BATS.Parser.States
              n87 = Select(t=w290, s=w289, f=w288) -> (s? t:f=w287:u8)
              n88 = Select(t=w292, s=w289, f=w291) -> (s? t:f=w285:T3)
            }
            frame True {
              w299 = u8 0  # t
              w301 = T3."Read.Sequenced.Unit.Header"  # t
              w300 = T3."Read.Msg"  # BATS.Parser.States
              n89 = call "compress.buffer.generated.vi"("start.idx"=w307, "buffer.length"=w308, "buffer"=w309) -> ("buffer.length.out"=w297:u8, "buffer.out"=w295:u64[])  [unwired: 7 in]
              n90 = To Unsigned Word Integer(number=w307) -> (unsigned 16bit integer=w305:u16)
              n91 = Add(x=w306, y=w305) -> (x+y=w293:u16)
              n92 = Greater Or Equal?(x=w293, y=w304) -> (x >= y?=w302:bool)
              n93 = Boolean To (0,1)(Boolean=w302) -> ()  [unwired: 1 out]
              n94 = Or(x=w303, y=w302) -> (x .or. y?=w298:bool)
              n95 = Select(t=w301, s=w298, f=w300) -> (s? t:f=w294:T3)
              n96 = Select(t=w299, s=w298, f=w297) -> (s? t:f=w296:u8)
            }
          }
          n97 = case shown="True" w233 {
            tunnel: w240 -> [w261 w282]
            tunnel: w239 -> [w262 w283]
            tunnel: w238 -> [_ w267]
            tunnel: [w261 w264] -> w237
            tunnel: [w260 w263] -> w215
            frame False {
              n98 = Unbundle(w262) -> ("Next.Seq.No"=w260:u32)  [unwired: 17 out]
            }
            frame True {
              # "Message Ready"
              n99 = Unbundle(w283) -> ("Next.Seq.No"=w265:u32)  [unwired: 17 out]
              n100 = Unbundle(w282) -> ("type"=w281:T8, "side"=w280:u8, "orderId"=w279:u64, "quantity"=w278:u32, "symbol"=w277:u64, "price"=w276:u64, "executed.qty"=w275:u32, "canceled.qty"=w274:u32, "remaining.qty"=w273:u32, "seconds"=w272:u64, "nanoseconds"=w271:u64, "Add"=w270:bool, "Edit"=w269:bool, "Remove"=w268:bool)  [unwired: 3 out]
              n101 = Increment(x=w265) -> (x+1=w263:u32)
              n102 = Bundle(cluster=w282, "type"=w281, "side"=w280, "orderId"=w279, "quantity"=w278, "symbol"=w277, "price"=w276, "executed.qty"=w275, "canceled.qty"=w274, "remaining.qty"=w273, "seconds"=w272, "nanoseconds"=w271, "Add"=w270, "Edit"=w269, "Remove"=w268, "seq no"=w265, "recv.time"=w267, "parse.time"="time") -> (w264:T7)
            }
          }
          n103 = Bundle By Name(cluster=w241, "write"=w233, "data"=w242) -> (w214:cluster{"write":bool, "data":u64[]})
          n104 = Unbundle(w232) -> ("Saved.BATS.Parser.State"=w230:T3, "Hdr Length (U16)"=w229:u16, "MessageLength (U8)"=w228:u8, "MessageType (U8)"=w227:u8, "Time (U32)"=w226:u32, "Message Counter (U8)"=w224:u8, "i"=w223:u16, "Number.of.Tickers"=w222:u16, "n"=w221:u16, "msg.counter"=w220:u8, "msg.length"=w219:u8, "buffer.start"=w218:u8)  [unwired: 6 out]
          n105 = Bundle(cluster=w232, "BATS.Parser.States"=w231, "Saved.BATS.Parser.State"=w230, "Hdr Length (U16)"=w229, "MessageLength (U8)"=w228, "MessageType (U8)"=w227, "Time (U32)"=w226, "Total Counter (U16)"=w225, "Message Counter (U8)"=w224, "i"=w223, "Number.of.Tickers"=w222, "n"=w221, "msg.counter"=w220, "msg.length"=w219, "buffer.start"=w218, "buffer.length"=w217, "buffer"=w216, "Next.Seq.No"=w215, "debug"=w214) -> (w213:T4)
          n106 = To Variant(anything=w237) -> (Variant=w234:variant)
          n107 = call "FIFO.WRITE.vi"("FIFO Name"=w236, "Data Type"=w235, "Element"=w234, "Input Valid"=w233) -> ()  [unwired: 10 in, 2 out]
        }
      }
    }
  }
  "Ready.for.Udp.Input" <- w1
  n108 = Unbundle(w8) -> ("debug"=w7:cluster{"write":bool, "data":u64[]})  [unwired: 17 out]
  n109 = Unbundle(w8) -> ("BATS.Parser.States"=w27:T3, "Saved.BATS.Parser.State"=w26:T3, "Hdr Length (U16)"=w25:u16, "MessageLength (U8)"=w24:u8, "MessageType (U8)"=w23:u8, "Time (U32)"=w22:u32, "Total Counter (U16)"=w21:u16, "Message Counter (U8)"=w20:u8, "i"=w19:u16, "Number.of.Tickers"=w18:u16, "n"=w17:u16, "msg.counter"=w16:u8, "msg.length"=w15:u8, "buffer.start"=w14:u8, "buffer.length"=w13:u8, "buffer"=w12:u64[], "Next.Seq.No"=w11:u32, "debug"=w30:cluster{"write":bool, "data":u64[]})
  n110 = Unbundle(w7) -> ("write"=w2:bool, "data"=w6:u64[])
  n111 = Unbundle(w30) -> ("data"=w28:u64[])  [unwired: 1 out]
  n112 = Bundle(cluster=w30, "write"=w29, "data"=w28) -> (w10:cluster{"write":bool, "data":u64[]})
  n113 = To Variant(anything=w6) -> (Variant=w3:variant)
  n114 = call "FIFO.WRITE.vi"("FIFO Name"=w5, "Data Type"=w4, "Element"=w3, "Input Valid"=w2) -> ()  [unwired: 10 in, 2 out]
  n115 = Bundle(cluster=w8, "BATS.Parser.States"=w27, "Saved.BATS.Parser.State"=w26, "Hdr Length (U16)"=w25, "MessageLength (U8)"=w24, "MessageType (U8)"=w23, "Time (U32)"=w22, "Total Counter (U16)"=w21, "Message Counter (U8)"=w20, "i"=w19, "Number.of.Tickers"=w18, "n"=w17, "msg.counter"=w16, "msg.length"=w15, "buffer.start"=w14, "buffer.length"=w13, "buffer"=w12, "Next.Seq.No"=w11, "debug"=w10) -> (w9:T4)
  n116 = feedback-in #1(w9) -> ()
